vi "Read.vi"(8 "error in (no error)":errorcluster, 10 "byte count":u32, 11 "Serial Logging Decorator in":refnum<class "Serial Logging Decorator.lvclass">) -> (0 "error out":errorcluster, 2 "read buffer":string, 3 "Serial Logging Decorator out":refnum<class "Serial Logging Decorator.lvclass">)   [LabVIEW 2020, in "Serial Logging Decorator.lvclass"]
uses:
  Serial Logging Decorator.lvclass
  Serial Logging Decorator.lvclass/Serial Logging Decorator.ctl
  Log/Log.lvclass
  Serial/Serial.lvclass/Serial.lvclass
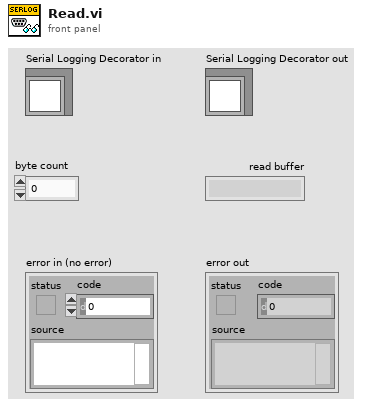
[diagram p1: front panel]
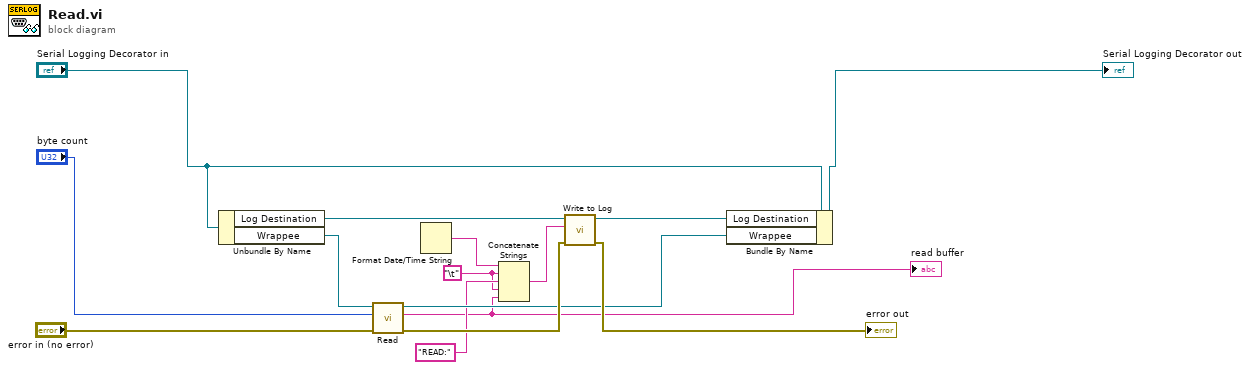
[diagram p0: block diagram]
diagram:
  w2 = "\t" ("string")
  n1 = Unbundle By Name("Serial Logging Decorator in") -> ("Log Destination"=w15:refnum<class "Log.lvclass">, "Wrappee"=w6:refnum<class "Serial.lvclass">)
  n2 = call-dynamic "Read.vi"("error in (no error)"="error in (no error)", "byte count"="byte count", "Serial in"=w6) -> ("error out"=w7:errorcluster, "read buffer"=w1:string, "Serial out"=w5:refnum<class "Serial.lvclass">)  [unwired: 6 in]
  "read buffer" <- w1
  n3 = Format Date/Time String() -> (date/time string=w13:string)  [unwired: 3 in]
  n4 = Concatenate Strings(w13, w2, "READ:", w2, w1) -> (w12:string)
  n5 = call-dynamic "Write to Log.vi"("error in (no error)"=w7, "Text to Write"=w12, "Log in"=w15) -> ("error out"=→"error out":errorcluster, "Log out"=w14:refnum<class "Log.lvclass">)  [unwired: 7 in]
  n6 = Bundle By Name(cluster="Serial Logging Decorator in", "Log Destination"=w14, "Wrappee"=w5) -> (→"Serial Logging Decorator out":refnum<class "Serial Logging Decorator.lvclass">)
